vi "GetTerms4.vi"(0 "XRef":T12, 1 "State In":T10) -> (14 "Terms":T2, 15 "Fatal Error Out":T1)   [LabVIEW 2021, in "FirstXNode .xnode"]
uses:
  FirstXNode .xnode
  <vilib>/XNodeSupport/XNodeXNodeRef.ctl
  State.ctl
  <vilib>/XNodeSupport/XNodeBounds.ctl
  <vilib>/XNodeSupport/XNodeInt.ctl
  <vilib>/XNodeSupport/XNodeTerm4Array.ctl
  <vilib>/XNodeSupport/XNodeTerm4.ctl
  <vilib>/XNodeSupport/XNodeString.ctl
  <vilib>/XNodeSupport/XNodeVariant.ctl
  <vilib>/XNodeSupport/XNodeRect32.ctl
  <vilib>/XNodeSupport/XNodeBool.ctl
  <vilib>/XNodeSupport/XNodeTermDirection.ctl
  <vilib>/XNodeSupport/XNodeErrorCluster.ctl
  <vilib>/XNodeSupport/NI_XNodeSupport.lvlib
  <vilib>/Utility/Data Type/NI_Data Type.lvlib
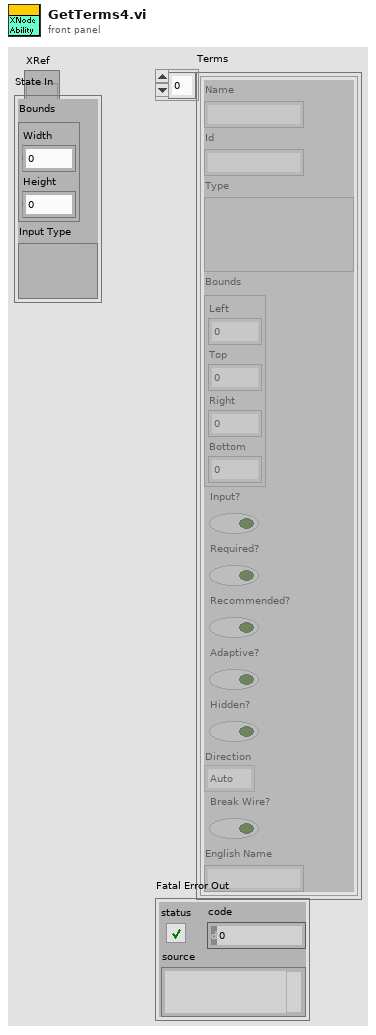
[diagram p1: front panel]
types:
  T1 = typedef "NI_XNodeSupport.lvlib/XNodeErrorCluster.ctl" = errorcluster
  T2 = typedef "NI_XNodeSupport.lvlib/XNodeTerm4Array.ctl" = T3[]
  T3 = typedef "NI_XNodeSupport.lvlib/XNodeTerm4.ctl" = cluster{"Name":T4, "Id":T4, "Type":T5, "Bounds":T6, "Input?":T8, "Required?":T8, "Recommended?":T8, "Adaptive?":T8, "Hidden?":T8, "Direction":T9, "Break Wire?":T8, "English Name":T4}
  T4 = typedef "NI_XNodeSupport.lvlib/XNodeString.ctl" = string
  T5 = typedef "NI_XNodeSupport.lvlib/XNodeVariant.ctl" = variant
  T6 = typedef "NI_XNodeSupport.lvlib/XNodeRect32.ctl" = cluster{"Left":T7, "Top":T7, "Right":T7, "Bottom":T7}
  T7 = typedef "NI_XNodeSupport.lvlib/XNodeInt.ctl" = i32
  T8 = typedef "NI_XNodeSupport.lvlib/XNodeBool.ctl" = bool
  T9 = typedef "NI_XNodeSupport.lvlib/XNodeTermDirection.ctl" = enum32{"Auto", "Up", "Down", "Left", "Right", "Center"}
  T10 = typedef "FirstXNode .xnode/State.ctl" = cluster{"Bounds":T11, "Input Type":variant}
  T11 = typedef "NI_XNodeSupport.lvlib/XNodeBounds.ctl" = cluster{"Width":T7, "Height":T7}
  T12 = typedef "NI_XNodeSupport.lvlib/XNodeXNodeRef.ctl" = refnum<vi>
  T13 = typedef "NI_Data Type.lvlib/Data Type.ctl" = enum8{"Invalid Type", "Void", "I8", "I16", "I32", "I64", "U8", "U16", "U32", "U64", "Single Float", "Double Float", "Extended Float", "Single Complex", "Double Complex", "Extended Complex", "Enum U8", "Enum U16", "Enum U32", "Enum U64", "Single Float With Unit", "Double Float With Unit", "Extended Float With Unit", "Single Complex with Unit", "Double Complex with Unit", "Extended Complex with Unit", "Boolean", "String", "Path", "Picture", "Tag", "Array", "Cluster", "Variant", "LV Variant", "Waveform", "Timestamp", "Digital Waveform", "Digital Data", "ExpressData", "Refnum", "External Data", "VI", "Poly VI", "LabVIEW Class Instance", "Fixed Point", "Set Collection", "Map Collection"}
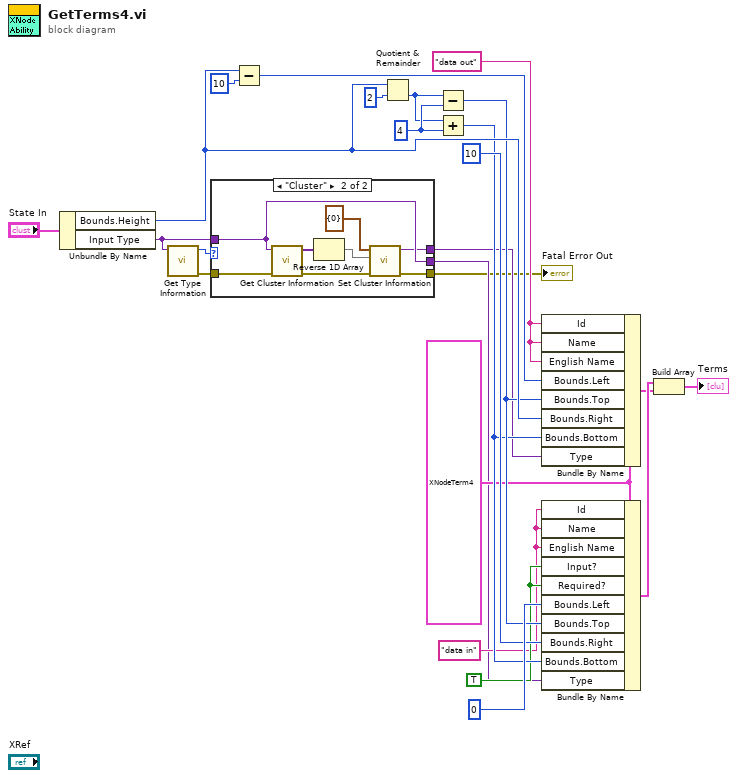
[diagram p0: block diagram]
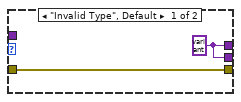
[diagram p2: hidden frame]
diagram:
  w7 = "data out"
  w9 = "data in"
  w10 = TRUE
  w22 = T7 4 ("y")
  w8 = T3 {"Name"="", "Id"="", "Type"=variant, "Bounds"={"Left"=0, "Top"=0, "Right"=0, "Bottom"=0}, "Input?"=FALSE, "Required?"=FALSE, "Recommended?"=FALSE, "Adaptive?"=FALSE, "Hidden?"=FALSE, "Direction"=enum."Auto", "Break Wire?"=FALSE, "English Name"=""} ("Term 4")
  n1 = Unbundle By Name("State In") -> ("Bounds.Height"=w16:T7, "Input Type"=w5:variant)
  n2 = call <vilib>:"Get Type Information.vi"("variant"=w5) -> ("error out"=w2:errorcluster, "type"=w6:T13)  [unwired: 6 in, 3 out]
  n3 = case shown="\"Cluster\"" w6 {
    tunnel: w5 -> [_ w34]
    tunnel: [w26 w34] -> w4
    tunnel: [w26 w32] -> w3
    tunnel: w2 -> [w25 w31]
    tunnel: [w25 w29] -> w1
    frame "Invalid Type", Default {
      w26 = variant ("Input Type")
    }
    frame "Cluster" {
      n4 = call <vilib>:"Get Cluster Information.vi"("error in (no error)"=w31, "variant"=w34) -> ("error out"=w30:errorcluster, "cluster elements"=w28:variant[])  [unwired: 8 in]
      n5 = Reverse 1D Array(array=w28) -> (reversed array=w27:variant[])
      n6 = call <vilib>:"Set Cluster Information.vi"("error in (no error)"=w30, "Cluster Elements"=w27, "Variant in"=cluster{i32} {0}) -> ("error out"=w29:errorcluster, "Variant out"=w32:variant)  [unwired: 7 in]
    }
  }
  "Fatal Error Out" <- w1
  n7 = Subtract(x=w16, y=T7 10 ("Bounds.Right")) -> (x-y=w14:T7)
  n8 = Quotient & Remainder(x=w16, y=T7 2) -> (floor(x/y)=w17:T7)  [unwired: 1 out]
  n9 = Subtract(x=w17, y=w22) -> (x-y=w13:T7)
  n10 = Add(x=w17, y=w22) -> (x+y=w12:T7)
  n11 = Bundle By Name(cluster=w8, "Id"=w7, "Name"=w7, "English Name"=w7, "Bounds.Left"=w14, "Bounds.Top"=w13, "Bounds.Right"=w16, "Bounds.Bottom"=w12, "Type"=w3) -> (w11:T3)
  n12 = Bundle By Name(cluster=w8, "Id"=w9, "Name"=w9, "English Name"=w9, "Input?"=w10, "Required?"=w10, "Bounds.Left"=T7 0, "Bounds.Top"=w13, "Bounds.Right"=T7 10, "Bounds.Bottom"=w12, "Type"=w4) -> (w20:T3)
  n13 = Build Array(w20, w11) -> (→"Terms":T3[])
